vi "Enable.vi"(11 "logger in":refnum<class "Logger.lvclass">) -> (3 "logger out":refnum<class "Logger.lvclass">)   [LabVIEW 2018, in "GLog.lvlib" / "Logger.lvclass"]
uses:
  Logger.lvclass
  Logger.lvclass/Logger.ctl
panel:
  # "Connector Pane"
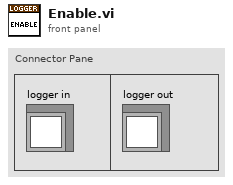
[diagram p1: front panel]
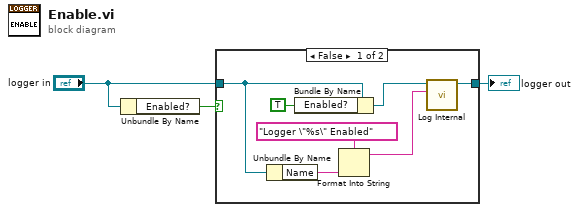
[diagram p0: block diagram]
diagram:
  n1 = Unbundle By Name("logger in") -> ("Enabled?"=w2:bool)
  n2 = case shown="False" w2 {
    tunnel: "logger in" -> [w10 w11]
    tunnel: [w9 w11] -> w3
    frame False {
      n3 = Unbundle By Name(w10) -> ("Name"=w6:string)
      n4 = Bundle By Name(cluster=w10, "Enabled?"=TRUE) -> (w8:refnum<class "Logger.lvclass">)
      n5 = Format Into String(format string="Logger \"%s\" Enabled" ("message"), w6) -> (resulting string=w4:string)  [unwired: 2 in, 1 out]
      n6 = call "Log Internal.vi"("message"=w4, "logger in"=w8) -> ("logger out"=w9:refnum<class "Logger.lvclass">)  [unwired: 9 in]
    }
    frame True {
    }
  }
  "logger out" <- w3
